vi "thermal_optical_capture_14.vi"() -> ()   [LabVIEW 2025]
uses:
  VIs_needed/Grab Manager Mode.ctl
  <vilib>/vision/driver/IMAQdx.llb/IMAQdx Buffer Number Mode.ctl
  <vilib>/vision/driver/NI_Vision_Acquisition_Software.lvlib
  <resource>/objmgr/imaqdx.rc
panel:
  in  "Stop":bool
  out "Images Saved Per Second":dbl
  out "Images Behind":i32
  out "Images Acquired Per Second":dbl
  in  "Skip Count":u32
  out "Write Speed Waveform":dbl(graph) caption="Image File Write Speed"
  out "Times between Frames":u32
  in  "Number of Images":u32=30
  in  "Camera Name":refnum<k21> caption="IMAQdx Session"
  out "Thermal Preview":T1(plugin-control)
  in  "Stop Preview":bool
  out "Times bw Thermal Frames":u32
  in  "STOP ACQUISITION":bool
  in  "Focus":dbl(slide) scale=0.0..100.0
  out "Thermal Frame Out":string
  in  "Output Folder":path
  in  "thermal capture interval (s)":dbl
  in  "Flag Button":bool
  in  "Stop & Save":bool
  in  "Record":bool
  # "Thermal Record"
  # "(Enter \"28\")"
  # "^ append to base data folder \"...\\test_n\\raw\" for nth recording"
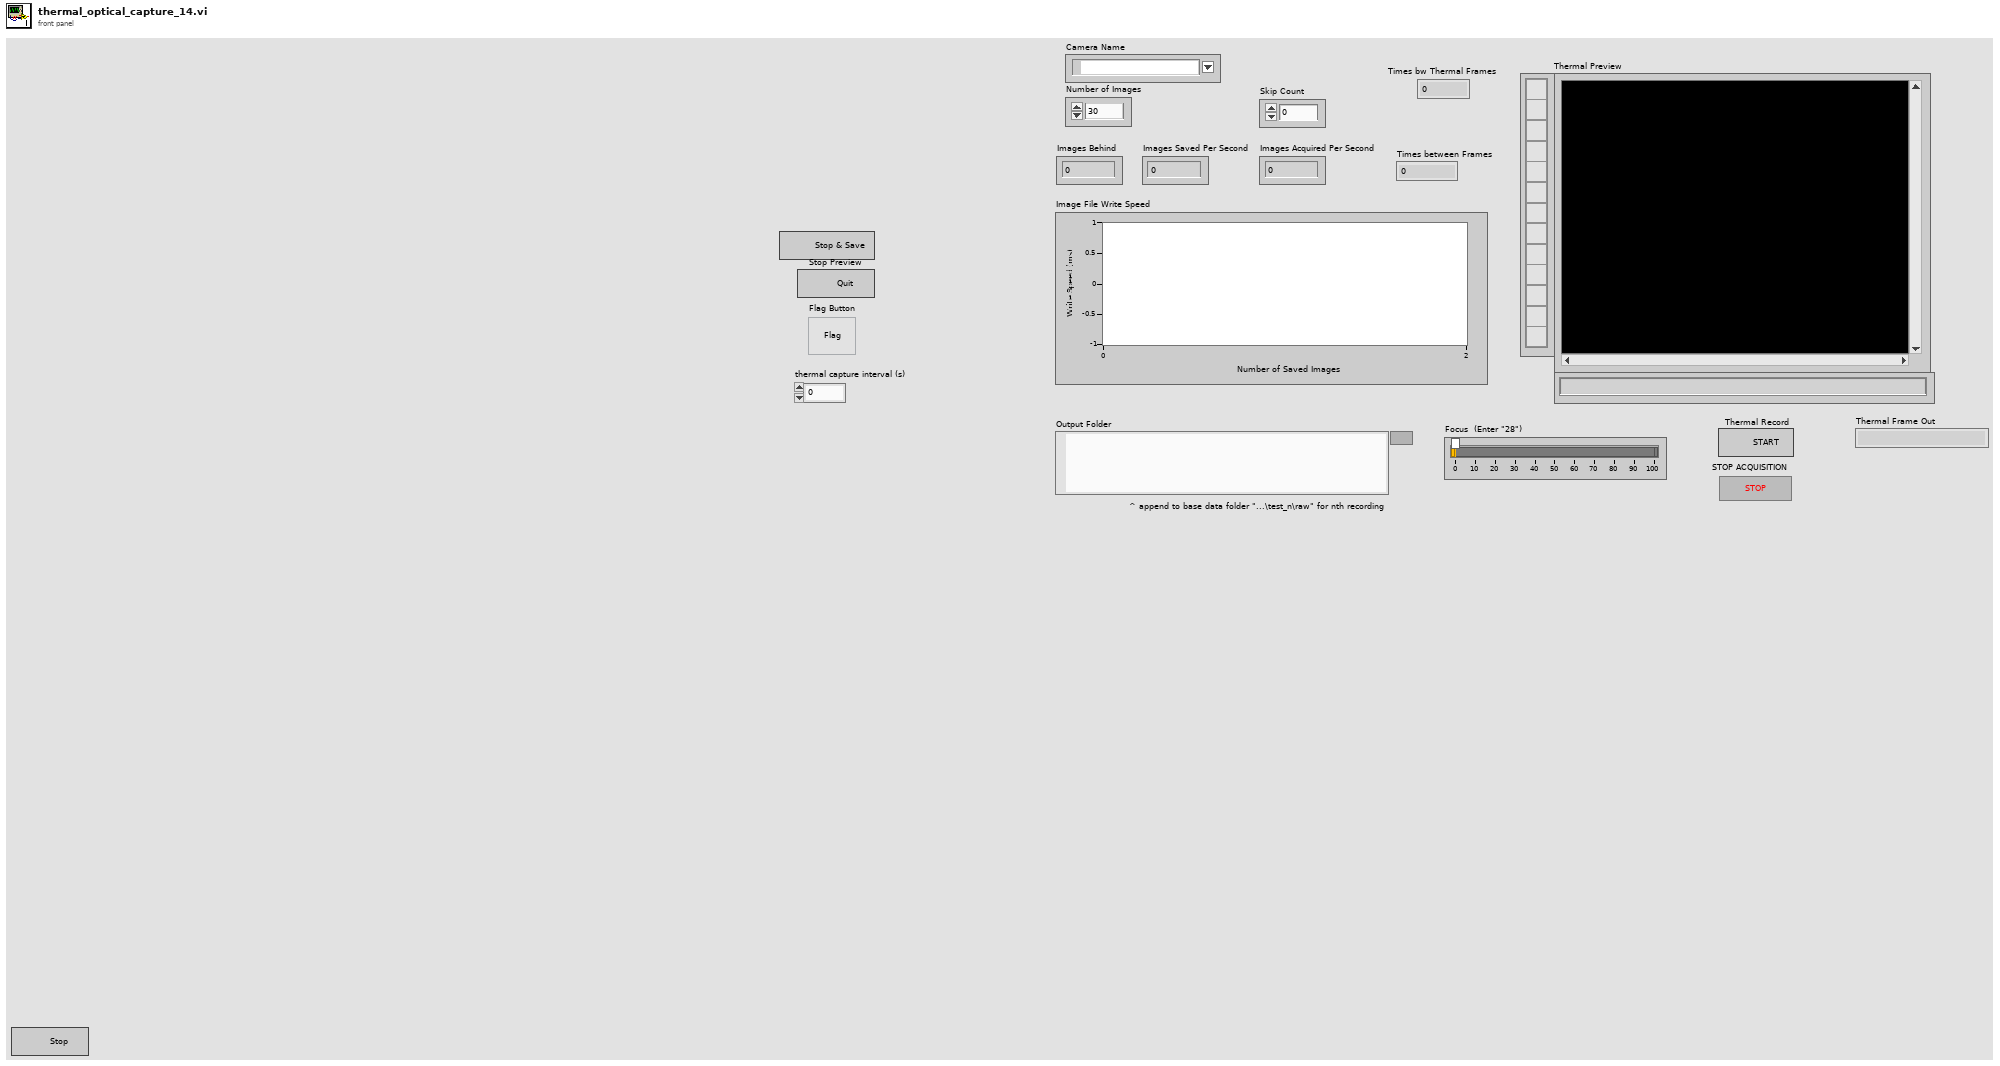
[diagram p1: front panel]
types:
  T1 = typedef "IMAQ Image.ctl" = refnum<image>
  T2 = typedef "Grab Manager Mode.ctl" = enum16{"Create Processing Images", "Lock", "Add Acquired Image", "Get Acquired Image", "Unlock", "Dispose Processing Images"}
  T3 = cluster{"Number of Processing Images":u32, "Image Border Size":u32}
  T4 = typedef "NI_Vision_Acquisition_Software.lvlib/IMAQdx Buffer Number Mode.ctl" = enum32{"Next", "Last", "Buffer Number", "Every", "Last New"}
  T5 = enum16{"open", "replace", "create", "open or create", "replace or create", "replace or create with confirmation"}
  T6 = enum16{"big-endian, network order", "native, host order", "little-endian"}
  T7 = typedef "Image Type" = u32
  T8 = typedef "IMAQdx.ctl" = refnum<k21>
  T9 = enum16{"Standard", "Buffered", "CRLF", "Immediate"}
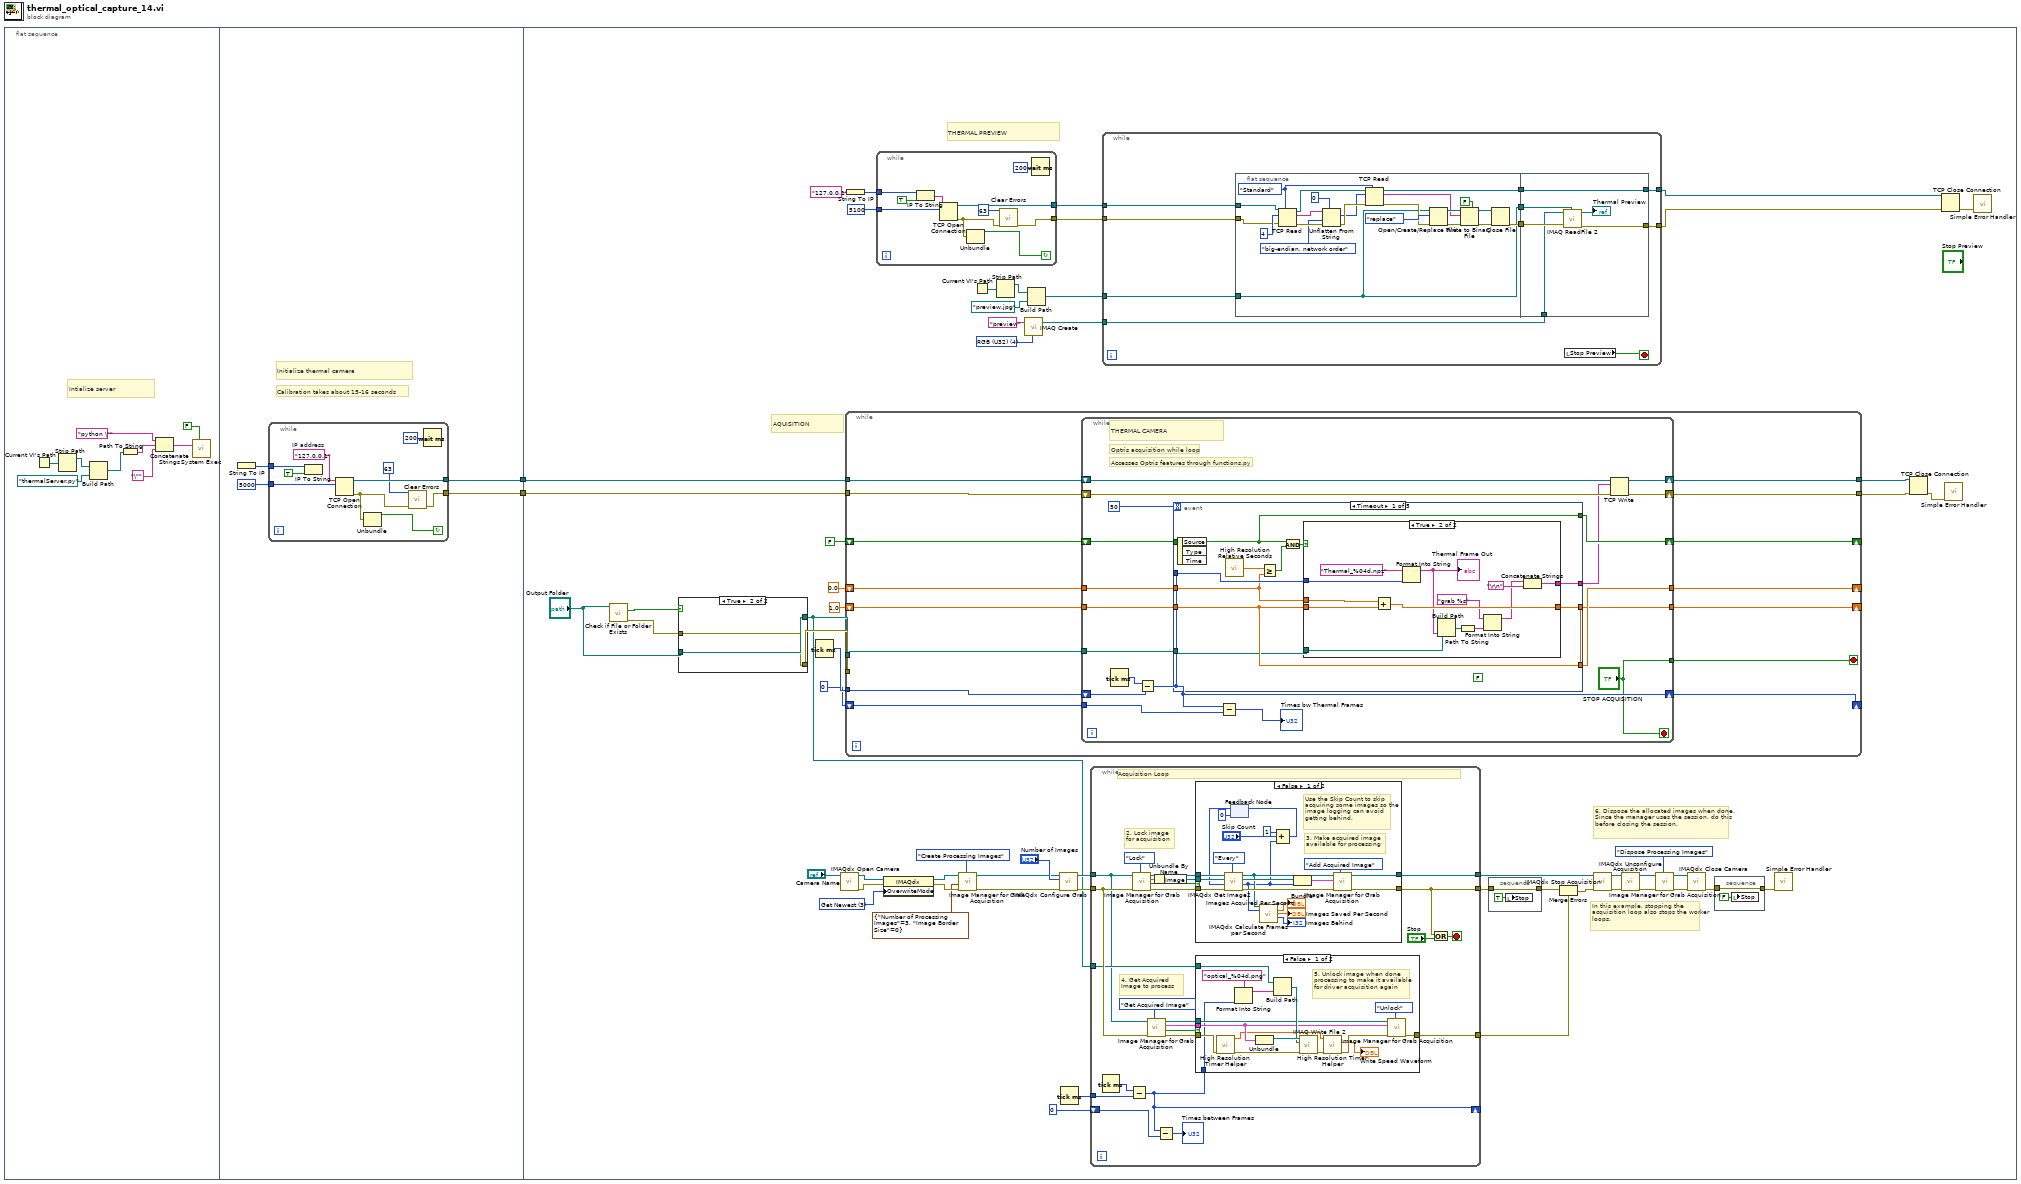
[diagram p0: block diagram]
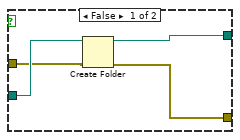
[diagram p4: hidden frame]
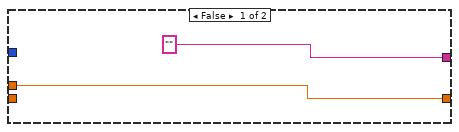
[diagram p5: hidden frame]
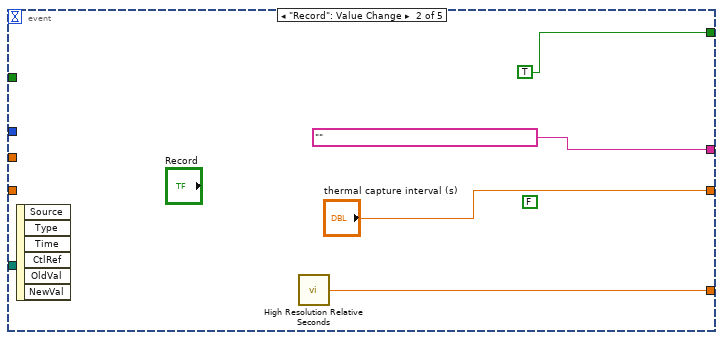
[diagram p6: hidden frame]
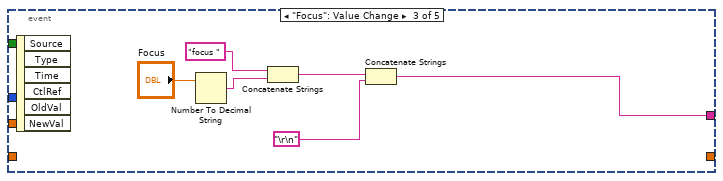
[diagram p7: hidden frame]
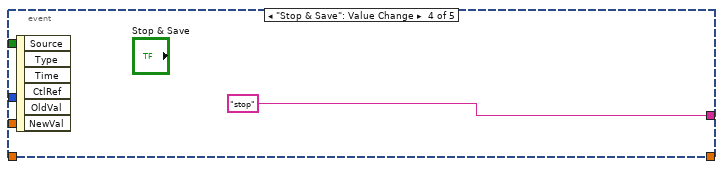
[diagram p8: hidden frame]
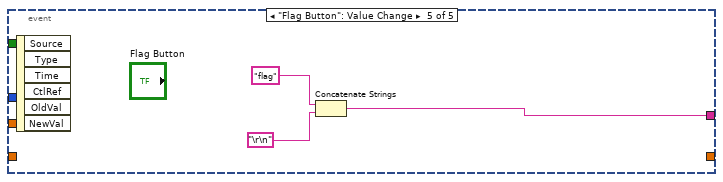
[diagram p9: hidden frame]
diagram:
  n1 = flat-sequence {
    tunnel: [w13] -> w2
    tunnel: [w12] -> w1
    tunnel: w1 -> [w81]
    tunnel: w2 -> [w80]
    frame #0 {
      # "Intialize server"
      n2 = Current VI's Path() -> (path=w6:path)
      n3 = Strip Path(path=w6) -> (stripped path=w7:path)  [unwired: 1 out]
      n4 = Build Path(base path=w7, name or relative path=path "thermalServer.py") -> (appended path=w4:path)
      n5 = Path To String(path=w4) -> (string=w10:string)
      n6 = Concatenate Strings("python \"" ("string"), w10, "\"" ("string")) -> (w9:string)
      n7 = call <vilib>:"System Exec.vi"("wait until completion? (T)"=FALSE, "command line"=w9) -> ()  [unwired: 6 in, 4 out]
    }
    frame #1 {
      # "Initialize thermal camera"
      # "Calibration takes about 15-16 seconds"
      n8 = String To IP() -> (0:w15:u32)  [unwired: 1 in]
      n9 = while {
        tunnel: [w20] -> w13
        tunnel: [w25] -> w12
        tunnel: w15 -> [w24]
        tunnel: u16 5000 ("remote port or service name") -> [w22]
        stop <- w17 continue-if-true
        w16 = "127.0.0.1"  # IP address
        n10 = IP To String(1:TRUE ("dot notation? (F)"), 2:w24) -> ()  [unwired: 1 out]
        n11 = TCP Open Connection(address=w16, remote port or service name=w22) -> (connection ID=w25:refnum<k5>, error out=w21:errorcluster)  [unwired: 3 in]
        n12 = Unbundle(w21) -> ("status"=w17:bool)  [unwired: 2 out]
        n13 = call <vilib>:"Clear Errors.vi"("error in (no error)"=w21, "specific error code to clear (0: all)"=63) -> ("error out"=w20:errorcluster)  [unwired: 4 in, 1 out]
        n14 = Wait (ms)(milliseconds to wait=u32 200) -> ()  [unwired: 1 out]
      }
    }
    frame #2 {
      w54 = u32 3 items=["Get Oldest"=0, "Fail"=2, "Get Newest"=3] ("OverwriteMode")
      w68 = T7 4 items=["Grayscale (U8)", "Grayscale (I16)", "Grayscale (SGL)", "Complex (CSG)", "RGB (U32)", "HSL (U32)", "RGB (U64)", "Grayscale (U16)"] ("Image Type")
      # "6. Dispose the allocated images when done. Since the manager uses the session, do this before closing the session."
      # "In this example, stopping the acquisition loop also stops the worker loops."
      # "THERMAL PREVIEW"
      # "AQUISITION"
      n15 = call <vilib>:"Check if File or Folder Exists.vi"("path"="Output Folder") -> ("error out"=w60:errorcluster, "file or folder exists?"=w62:bool)  [unwired: 8 in, 1 out]
      n16 = case shown="True" w62 {
        tunnel: "Output Folder" -> [w155 w157]
        tunnel: [w154 w157] -> w26
        tunnel: w60 -> [w153 w156]
        tunnel: [w152 w156] -> w59
        frame False {
          n17 = Create Folder(path (use dialog)=w155, error in=w153) -> (created path=w154:path, error out=w152:errorcluster)  [unwired: 1 in, 1 out]
        }
        frame True {
        }
      }
      n18 = Tick Count (ms)() -> (millisecond timer value=w76:u32)
      n19 = call <vilib>:"IMAQdx Open Camera.vi"("Session In"="Camera Name") -> ("error out"=w50:errorcluster, "Session Out"=w51:T8)  [unwired: 2 in, 7 out]
      n20 = while {
        tunnel: [w220] -> w82
        tunnel: [w219] -> w83
        tunnel: w81 -> [w218]
        tunnel: w80 -> [w217]
        shift-right: [w216] -> _
        shift-left: 0.0 -> [w213]
        shift-right: [w214] -> _
        shift-left: 1.0 -> [w211]
        shift-right: [w215] -> _
        shift-left: FALSE -> [w212]
        tunnel: w76 -> [w210]
        shift-right: [w207] -> _
        shift-left: u32 0 -> [w209]
        tunnel: w26 -> [w208]
        tunnel: w59 -> [_]
        stop <- w206 stop-if-true
        n21 = while {
          tunnel: [w235] -> w216
          tunnel: [w232] -> w214
          tunnel: w213 -> [w231]
          tunnel: w211 -> [w229]
          tunnel: w209 -> [w225]
          tunnel: w208 -> [w223]
          shift-right: [w238] -> w219
          shift-left: w218 -> [w237]
          shift-right: [w239] -> w220
          shift-left: w217 -> [w236]
          shift-right: [w233] -> w215
          shift-left: w212 -> [w230]
          shift-right: [w222] -> w207
          shift-left: w210 -> [w226]
          tunnel: ["STOP ACQUISITION"] -> w206
          stop <- "STOP ACQUISITION" stop-if-true
          # "THERMAL CAMERA"
          # "Optris acquisition while loop"
          # "Accesses Optris features through functions.py"
          n22 = Tick Count (ms)() -> (millisecond timer value=w227:u32)
          n23 = Subtract(x=w227, y=w226) -> (x-y=w222:u32)
          n24 = event shown="[0] Timeout" {
            selector: _ -> [_ _ _ _ _]
            dyn-events: _ -> [_ _ _ _ _]
            timeout: 50 -> [_ _ _ _ _]
            tunnel: [w245 "" w269 "stop" w278] -> w228
            tunnel: w222 -> [w246 _ _ _ _]
            tunnel: [w243 w268 _ _ _] -> w235
            tunnel: [w241 TRUE _ _ _] -> w233
            tunnel: [w242 "thermal capture interval (s)" _ _ _] -> w232
            tunnel: w231 -> [w244 _ _ _ _]
            tunnel: w230 -> [w241 _ _ _ _]
            tunnel: w229 -> [w242 _ _ _ _]
            tunnel: w223 -> [w240 _ _ _ _]
            event Timeout {
              (unwired) FALSE
              n25 = event-data() -> ()  [unwired: 1 in, 3 out]
              n26 = call <vilib>:"High Resolution Relative Seconds.vi"() -> ("relative seconds"=w249:dbl)
              n27 = Greater Or Equal?(x=w249, y=w244) -> (x >= y?=w248:bool)
              n28 = And(x=w241, y=w248) -> (x .and. y?=w247:bool)
              n29 = case shown="True" w247 {
                tunnel: w246 -> [_ w262]
                tunnel: ["" w263] -> w245
                tunnel: w244 -> [w250 w261]
                tunnel: w242 -> [_ w260]
                tunnel: [w250 w259] -> w243
                tunnel: w240 -> [_ w252]
                frame False {
                }
                frame True {
                  n30 = Add(x=w261, y=w260) -> (x+y=w259:dbl)
                  n31 = Format Into String(format string="Thermal_%04d.npz", w262) -> (resulting string=w253:string)  [unwired: 2 in, 1 out]
                  "Thermal Frame Out" <- w253
                  n32 = Build Path(base path=w252, name or relative path=w253) -> (appended path=w257:path)
                  n33 = Path To String(path=w257) -> (string=w255:string)
                  n34 = Format Into String(format string="grab %s", w255) -> (resulting string=w254:string)  [unwired: 2 in, 1 out]
                  n35 = Concatenate Strings(w254, "\r\n") -> (w263:string)
                }
              }
            }
            event "Record": Value Change {
              (unwired) FALSE
              n36 = event-data() -> ()  [unwired: 1 in, 6 out]
              n37 = call <vilib>:"High Resolution Relative Seconds.vi"() -> ("relative seconds"=w268:dbl)
            }
            event "Focus": Value Change {
              n38 = event-data() -> ()  [unwired: 1 in, 6 out]
              n39 = Number To Decimal String(number="Focus") -> (decimal integer string=w274:string)  [unwired: 1 in]
              n40 = Concatenate Strings("focus ", w274) -> (w271:string)
              n41 = Concatenate Strings(w271, "\r\n") -> (w269:string)
            }
            event "Stop & Save": Value Change {
              n42 = event-data() -> ()  [unwired: 1 in, 6 out]
            }
            event "Flag Button": Value Change {
              n43 = event-data() -> ()  [unwired: 1 in, 6 out]
              n44 = Concatenate Strings("flag", "\r\n") -> (w278:string)
            }
          }
          n45 = Subtract(x=w222, y=w225) -> (x-y=→"Times bw Thermal Frames":u32)
          n46 = TCP Write(connection ID=w237, data in=w228, error in (no error)=w236) -> (connection ID out=w238:refnum<k5>, error out=w239:errorcluster)  [unwired: 1 in, 1 out]
        }
      }
      n47 = String To IP(1:"127.0.0.1" ("name")) -> (0:w67:u32)
      n48 = while {
        tunnel: w67 -> [w167]
        tunnel: [w161] -> w66
        tunnel: [w165] -> w65
        tunnel: u16 5100 ("remote port or service name") -> [w163]
        stop <- w158 continue-if-true
        n49 = IP To String(1:TRUE ("dot notation? (F)"), 2:w167) -> (0:w166:string)
        n50 = TCP Open Connection(address=w166, remote port or service name=w163) -> (connection ID=w165:refnum<k5>, error out=w162:errorcluster)  [unwired: 3 in]
        n51 = Unbundle(w162) -> ("status"=w158:bool)  [unwired: 2 out]
        n52 = call <vilib>:"Clear Errors.vi"("error in (no error)"=w162, "specific error code to clear (0: all)"=63) -> ("error out"=w161:errorcluster)  [unwired: 4 in, 1 out]
        n53 = Wait (ms)(milliseconds to wait=u32 200) -> ()  [unwired: 1 out]
      }
      n54 = property class="IMAQdx"(reference=w51, error in=w50, "OverwriteMode"=w54) -> (reference out=w53:T8, error out=w52:errorcluster)
      n55 = call "Image Manager for Grab Acquisition.vi"("Mode"=Grab_Manager_Mode."Create Processing Images", "error in (no error)"=w52, "Init Settings"=T3 {"Number of Processing Images"=3, "Image Border Size"=0}, "Session In"=w53) -> ("error out"=w46:errorcluster, "Session Out"=w45:T8)  [unwired: 4 in, 2 out]
      n56 = Current VI's Path() -> (path=w73:path)
      n57 = Strip Path(path=w73) -> (stripped path=w74:path)  [unwired: 1 out]
      n58 = call "IMAQ Create"("Image Name"="preview", "Image Type"=w68) -> ("New Image"=w71:T1)  [unwired: 3 in, 1 out]
      n59 = Build Path(base path=w74, name or relative path=path "preview.jpg") -> (appended path=w72:path)
      n60 = call <vilib>:"IMAQdx Configure Grab.vi"("error in"=w46, "Number of Buffers"="Number of Images", "Session In"=w45) -> ("error out"=w29:errorcluster, "Session Out"=w30:T8)  [unwired: 7 in]
      n61 = Tick Count (ms)() -> (millisecond timer value=w28:u32)
      n62 = while {
        tunnel: w29 -> [w102]
        tunnel: w30 -> [w100]
        tunnel: [w109] -> w41
        tunnel: [w110] -> w40
        tunnel: w26 -> [w101]
        tunnel: [w99] -> w31
        tunnel: w28 -> [w92]
        shift-right: [w89] -> _
        shift-left: u32 0 -> [w90]
        stop <- w111 stop-if-true
        # "4. Get Acquired Image to process"
        # "2. Lock image for acquisition"
        # "Acquisition Loop"
        n63 = Tick Count (ms)() -> (millisecond timer value=w93:u32)
        n64 = Subtract(x=w93, y=w92) -> (x-y=w89:u32)
        n65 = call "Image Manager for Grab Acquisition.vi"("Mode"=Grab_Manager_Mode."Lock", "error in (no error)"=w102, "Session In"=w100) -> ("error out"=w105:errorcluster, "No Available Image"=w106:bool, "Image Settings Out"=w104:cluster{"Image":T1, "Buffer Number":u32}, "Session Out"=w107:T8)  [unwired: 5 in]
        n66 = call "Image Manager for Grab Acquisition.vi"("Mode"=Grab_Manager_Mode."Get Acquired Image", "error in (no error)"=w102, "Session In"=w100) -> ("error out"=w95:errorcluster, "No Available Image"=w97:bool, "Image Settings Out"=w96:cluster{"Image":T1, "Buffer Number":u32}, "Session Out"=w94:T8)  [unwired: 5 in]
        n67 = Unbundle By Name(w104) -> ("Image"=w103:T1)
        n68 = Subtract(x=w89, y=w90) -> (x-y=→"Times between Frames":u32)
        n69 = case shown="False" w106 {
          tunnel: [w141 w151] -> w109
          tunnel: [w140 w150] -> w110
          tunnel: w107 -> [w149 w151]
          tunnel: w105 -> [w148 w150]
          tunnel: w103 -> [w142 _]
          frame False {
            # "3. Make acquired image available for processing"
            # "Use the Skip Count to skip acquiring some images so the image logging can avoid getting behind."
            n70 = feedback #1(u32 0) -> (w131:u32)
            n71 = call <vilib>:"IMAQdx Get Image2.vi"("Buffer Number Mode (Next)"=IMAQdx_Buffer_Number_Mode."Every", "error in"=w148, "Buffer Number In"=w131, "Image In"=w142, "Session In"=w149) -> ("error out"=w144:errorcluster, "Buffer Number Out"=w135:u32, "Image Out"=w146:T1, "Session Out"=w139:T8)  [unwired: 3 in]
            n72 = call <vilib>:"IMAQdx Calculate Frames per Second.vi"("Session In"=w139, "Buffer Number"=w135) -> ("Acquired Frames per Second"=→"Images Acquired Per Second":dbl, "Processed Frames per Second"=→"Images Saved Per Second":dbl, "Images Behind"=→"Images Behind":i32)  [unwired: 7 in, 4 out]
            n73 = Compound Arithmetic op=ADD(u32 1 ("value"), "Skip Count", w135) -> (w132:u32)
            n74 = feedback-in #1(w132) -> ()
            n75 = Bundle("Image Out"=w146, "Buffer Number Out"=w135) -> (w145:cluster{"Image Out":T1, "Buffer Number Out":u32})  [unwired: 1 in]
            n76 = call "Image Manager for Grab Acquisition.vi"("Mode"=Grab_Manager_Mode."Add Acquired Image", "error in (no error)"=w144, "Image Settings In"=w145, "Session In"=w139) -> ("error out"=w140:errorcluster, "Session Out"=w141:T8)  [unwired: 4 in, 2 out]
          }
          frame True {
            # "The Lock function already has a delay inside when no images are available to prevent loop from going too fast and starving the worker threads from getting processing time."
            # "Write to disk operation is taking longer so images aren't added back to manager. Wait until there is an available image"
          }
        }
        n77 = case shown="False" w97 {
          tunnel: w95 -> [w119 w129]
          tunnel: w96 -> [w121 _]
          tunnel: [w123 w129] -> w99
          tunnel: w101 -> [w127 _]
          tunnel: w94 -> [w120 _]
          tunnel: w89 -> [w113 _]
          frame False {
            # "5. Unlock image when done processing to make it available for driver acquisition again"
            n78 = call "High Resolution Timer Helper.vi"("error in (no error)"=w119) -> ("error out"=w118:errorcluster, "Current Time"=w114:dbl)  [unwired: 8 in, 1 out]
            n79 = Format Into String(format string="optical_%04d.png", w113) -> (resulting string=w126:string)  [unwired: 2 in, 1 out]
            n80 = Unbundle(w121) -> ("Image"=w128:T1)  [unwired: 1 out]
            n81 = Build Path(base path=w127, name or relative path=w126) -> (appended path=w124:path)
            n82 = call-poly "IMAQ Write File 2"("error in (no error)"=w118, "File Path"=w124, "Image"=w128) -> ("error out"=w117:errorcluster)  [unwired: 7 in, 1 out]
            n83 = call "High Resolution Timer Helper.vi"("error in (no error)"=w117, "Previous Time"=w114) -> ("error out"=w116:errorcluster, "Time Difference (ms)"=→"Write Speed Waveform":dbl)  [unwired: 7 in, 1 out]
            n84 = call "Image Manager for Grab Acquisition.vi"("Mode"=Grab_Manager_Mode."Unlock", "error in (no error)"=w116, "Image Settings In"=w121, "Session In"=w120) -> ("error out"=w123:errorcluster)  [unwired: 4 in, 3 out]
          }
          frame True {
            # "No acquired images to process"
          }
        }
        n85 = Or(x=w110, y="Stop") -> (x .or. y?=w111:bool)
      }
      n86 = while {
        tunnel: w71 -> [w172]
        tunnel: [w173] -> w57
        tunnel: [w177] -> w56
        tunnel: w72 -> [w175]
        tunnel: w66 -> [w170]
        tunnel: w65 -> [w169]
        stop <- w168 stop-if-true
        n87 = flat-sequence {
          tunnel: w175 -> [w181]
          tunnel: [w183] -> w176
          tunnel: [w182] -> w174
          tunnel: [w181] -> w171
          tunnel: w170 -> [w179]
          tunnel: w169 -> [w178]
          tunnel: [w205] -> w177
          tunnel: w176 -> [w205]
          tunnel: w174 -> [w204]
          tunnel: [w203] -> w173
          tunnel: w172 -> [w202]
          tunnel: w171 -> [w201]
          frame #0 {
            w192 = T9."Standard" ("mode (standard)")
            n88 = TCP Read(connection ID=w178, bytes to read=4, error in (no error)=w179, 7:w192) -> (connection ID out=w195:refnum<k5>, data out=w180:string, error out=w198:errorcluster)  [unwired: 1 in]
            n89 = Unflatten From String(type=0, binary string=w180, byte order (0:big-endian, network order)=T6."big-endian, network order", error in (no error)=w198) -> (value=w193:i32, error out=w194:errorcluster)  [unwired: 1 in, 1 out]
            n90 = TCP Read(connection ID=w195, bytes to read=w193, error in (no error)=w194, 7:w192) -> (connection ID out=w183:refnum<k5>, data out=w188:string, error out=w190:errorcluster)  [unwired: 1 in]
            n91 = Open/Create/Replace File(file path (use dialog)=w181, error in=w190, operation (0:open)=T5."replace") -> (refnum out=w189:refnum<file>, error out=w186:errorcluster)  [unwired: 3 in, 1 out]
            n92 = Write to Binary File(file (use dialog)=w189, data=w188, error in=w186, 5:FALSE ("prepend array or string size? (T)")) -> (refnum out=w184:refnum<file>, error out=w185:errorcluster)  [unwired: 2 in, 1 out]
            n93 = Close File(refnum=w184, error in=w185) -> (error out=w182:errorcluster)  [unwired: 1 out]
          }
          frame #1 {
            n94 = call "IMAQ ReadFile 2"("File Path"=w201, "error in (no error)"=w204, "Image"=w202) -> ("error out"=w203:errorcluster, "Image Out"=→"Thermal Preview":T1)  [unwired: 4 in, 3 out]
          }
        }
        n95 = local read "Stop Preview"() -> (w168:bool)
      }
      n96 = stacked-sequence {
        tunnel: [w87] -> w39
        tunnel: w40 -> [w87]
        frame #0 {
          n97 = local write "Stop"(TRUE ("Stop")) -> ()
        }
      }
      n98 = Merge Errors(w39, w31) -> (w42:errorcluster)
      n99 = call <vilib>:"IMAQdx Stop Acquisition.vi"("error in"=w42, "Session In"=w41) -> ("error out"=w43:errorcluster, "Session Out"=w44:T8)  [unwired: 8 out]
      n100 = call <vilib>:"IMAQdx Unconfigure Acquisition.vi"("error in"=w43, "Session In"=w44) -> ("error out"=w36:errorcluster, "Session Out"=w37:T8)  [unwired: 8 out]
      n101 = call "Image Manager for Grab Acquisition.vi"("Mode"=Grab_Manager_Mode."Dispose Processing Images", "error in (no error)"=w36, "Session In"=w37) -> ("error out"=w33:errorcluster, "Session Out"=w34:T8)  [unwired: 5 in, 2 out]
      n102 = call <vilib>:"IMAQdx Close Camera.vi"("error in"=w33, "Session In"=w34) -> ("error out"=w32:errorcluster)  [unwired: 9 out]
      n103 = stacked-sequence {
        tunnel: [w85] -> w38
        tunnel: w32 -> [w85]
        frame #0 {
          n104 = local write "Stop"(FALSE ("Stop")) -> ()
        }
      }
      n105 = call <vilib>:"Simple Error Handler.vi"("error in (no error)"=w38) -> ()  [unwired: 4 in, 5 out]
      n106 = TCP Close Connection(connection ID=w83, error in (no error)=w82) -> (error out=w84:errorcluster)  [unwired: 1 in, 1 out]
      n107 = TCP Close Connection(connection ID=w56, error in (no error)=w57) -> (error out=w58:errorcluster)  [unwired: 1 in, 1 out]
      n108 = call <vilib>:"Simple Error Handler.vi"("error in (no error)"=w84) -> ()  [unwired: 4 in, 5 out]
      n109 = call <vilib>:"Simple Error Handler.vi"("error in (no error)"=w58) -> ()  [unwired: 4 in, 5 out]
    }
  }
